vi "test request state rounds.vi"(8 "error in (no error)":errorcluster) -> (0 "error out":errorcluster, 3 "body":string)   [LabVIEW 2020, in "MCP Server tests.lvlib"]
doc: "Multi round-trip requests of MCP 2026-07-28 with requestState. fake_tool_two_questions asks the key first (Ask User.vi, a name) and in a later round the key second (Confirm With User.vi). Round 1 (id 70) is answered input_required with inputRequests.first and a requestState mcp-rs-...; round 2 (id 701) sends inputResponses first accept name Ada with that requestState and is answered input_required with inputRequests.second and a new requestState; round 3 (id 702) sends only the answer to second with the new requestState - the server carries the answer to first across the rounds - and the result is complete with name Ada and stored TRUE. The requests are sent with the LabVIEW HTTP Client directly."
uses:
  MCP Server tests.lvlib
  <vilib>/JDP Science/JSONtext/Next JSON Value.vi
  <vilib>/JDP Science/JSONtext/String Subset.vi
  <vilib>/JDP Science/JSONtext/Parsing/Advance past next JSON Value (inlined COPY).vi
  <vilib>/JDP Science/JSONtext/Parsing/Advance past whitespace.vi
  <vilib>/JDP Science/JSONtext/Parsing/Advance past String.vi
  <vilib>/JDP Science/JSONtext/Parsing/Advance past Number.vi
  <vilib>/JDP Science/JSONtext/Parsing/Advance past Line Ending.vi
  <vilib>/JDP Science/JSONtext/Parsing/Parse Full Path or Item Name.vi
  <vilib>/JDP Science/JSONtext/Parsing/Advance past Array.vi
  <vilib>/JDP Science/JSONtext/Parsing/Advance past Object.vi
  <vilib>/JDP Science/JSONtext/support/Error Cluster From Code.vi
  <vilib>/JDP Science/JSONtext/Offset/Find Item Locations by Path.vi
  <vilib>/addons/_JKI Toolkits/Caraya/classes/Test/Test.lvclass
  <vilib>/JDP Science/JSONtext/JSONtext.lvlib
  <vilib>/addons/_JKI Toolkits/Caraya/classes/Assert/Assert.lvclass
panel:
  out "lookup error":errorcluster
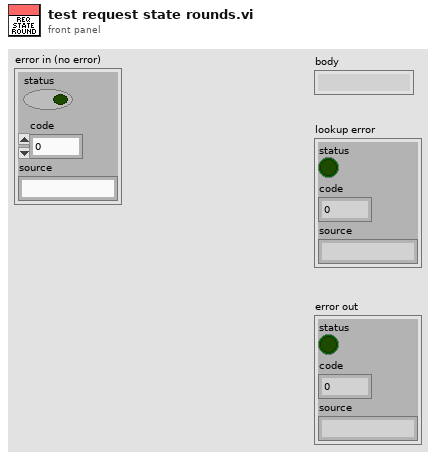
[diagram p1: front panel]
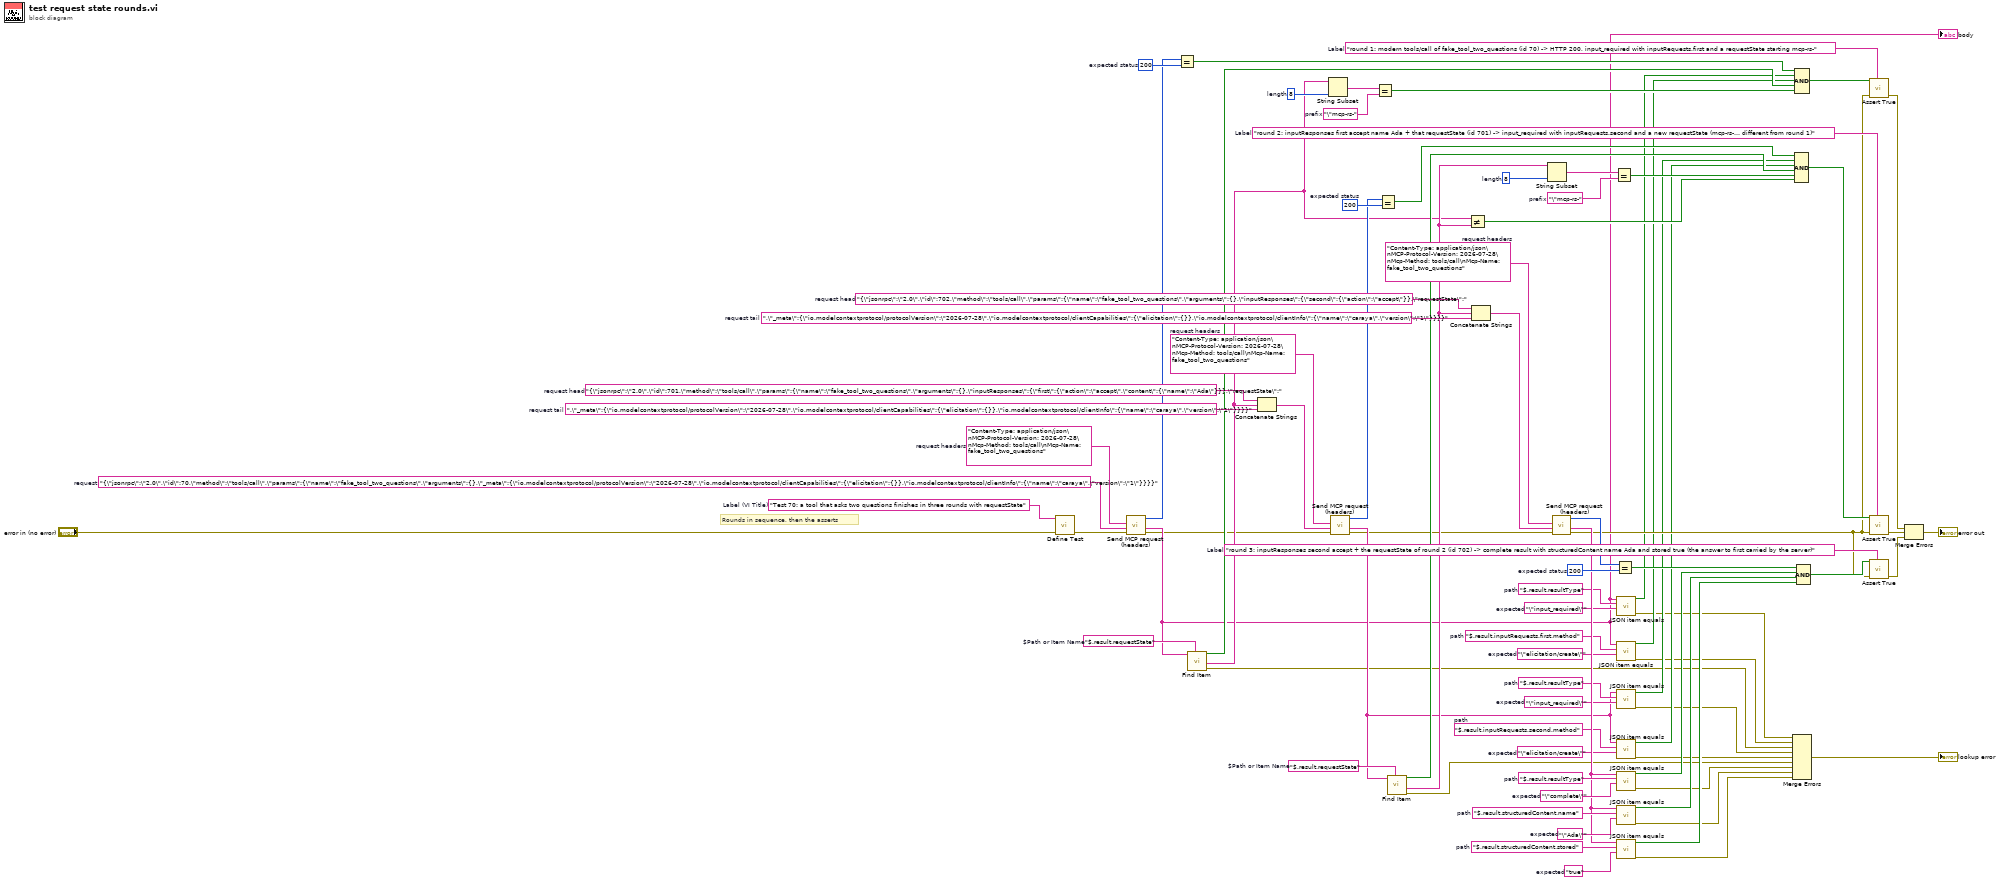
[diagram p0: block diagram]
diagram:
  w81 = "round 3: inputResponses second accept + the requestState of round 2 (id 702) -> complete result with structuredContent name Ada and stored true (the answer to first carried by the server)"  # Label
  w78 = "round 2: inputResponses first accept name Ada + that requestState (id 701) -> input_required with inputRequests.second and a new requestState (mcp-rs-… different from round 1)"  # Label
  w75 = "round 1: modern tools/call of fake_tool_two_questions (id 70) -> HTTP 200, input_required with inputRequests.first and a requestState starting mcp-rs-"  # Label
  w71 = "true"  # expected
  w70 = "$.result.structuredContent.stored"  # path
  w67 = "\"Ada\""  # expected
  w66 = "$.result.structuredContent.name"  # path
  w63 = "\"complete\""  # expected
  w62 = "$.result.resultType"  # path
  w60 = 200  # expected status
  w56 = "Content-Type: application/json\nMCP-Protocol-Version: 2026-07-28\nMcp-Method: tools/call\nMcp-Name: fake_tool_two_questions"  # request headers
  w54 = ",\"_meta\":{\"io.modelcontextprotocol/protocolVersion\":\"2026-07-28\",\"io.modelcontextprotocol/clientCapabilities\":{\"elicitation\":{}},\"io.modelcontextprotocol/clientInfo\":{\"name\":\"caraya\",\"version\":\"1\"}}}}"  # request tail
  w53 = "{\"jsonrpc\":\"2.0\",\"id\":702,\"method\":\"tools/call\",\"params\":{\"name\":\"fake_tool_two_questions\",\"arguments\":{},\"inputResponses\":{\"second\":{\"action\":\"accept\"}},\"requestState\":"  # request head
  w49 = 8  # length
  w48 = "\"mcp-rs-"  # prefix
  w44 = "$.result.requestState"  # $Path or Item Name
  w41 = "\"elicitation/create\""  # expected
  w40 = "$.result.inputRequests.second.method"  # path
  w37 = "\"input_required\""  # expected
  w36 = "$.result.resultType"  # path
  w34 = 200  # expected status
  w30 = "Content-Type: application/json\nMCP-Protocol-Version: 2026-07-28\nMcp-Method: tools/call\nMcp-Name: fake_tool_two_questions"  # request headers
  w28 = ",\"_meta\":{\"io.modelcontextprotocol/protocolVersion\":\"2026-07-28\",\"io.modelcontextprotocol/clientCapabilities\":{\"elicitation\":{}},\"io.modelcontextprotocol/clientInfo\":{\"name\":\"caraya\",\"version\":\"1\"}}}}"  # request tail
  w27 = "{\"jsonrpc\":\"2.0\",\"id\":701,\"method\":\"tools/call\",\"params\":{\"name\":\"fake_tool_two_questions\",\"arguments\":{},\"inputResponses\":{\"first\":{\"action\":\"accept\",\"content\":{\"name\":\"Ada\"}}},\"requestState\":"  # request head
  w24 = 8  # length
  w23 = "\"mcp-rs-"  # prefix
  w19 = "$.result.requestState"  # $Path or Item Name
  w16 = "\"elicitation/create\""  # expected
  w15 = "$.result.inputRequests.first.method"  # path
  w12 = "\"input_required\""  # expected
  w11 = "$.result.resultType"  # path
  w9 = 200  # expected status
  w5 = "Content-Type: application/json\nMCP-Protocol-Version: 2026-07-28\nMcp-Method: tools/call\nMcp-Name: fake_tool_two_questions"  # request headers
  w4 = "{\"jsonrpc\":\"2.0\",\"id\":70,\"method\":\"tools/call\",\"params\":{\"name\":\"fake_tool_two_questions\",\"arguments\":{},\"_meta\":{\"io.modelcontextprotocol/protocolVersion\":\"2026-07-28\",\"io.modelcontextprotocol/clientCapabilities\":{\"elicitation\":{}},\"io.modelcontextprotocol/clientInfo\":{\"name\":\"caraya\",\"version\":\"1\"}}}}"  # request
  w2 = "Test 70: a tool that asks two questions finishes in three rounds with requestState"  # Label (VI Title)
  # "Rounds in sequence, then the asserts"
  n1 = call <vilib>:"Define Test.vi"("error in (no error)"="error in (no error)", "Label (VI Title)"=w2) -> ("error out"=w3:errorcluster)  [unwired: 8 in, 1 out]
  n2 = call "Send MCP request (headers).vi"("error in (no error)"=w3, "request"=w4, "request headers"=w5) -> ("error out"=w6:errorcluster, "response"=w7:string, "status code"=w8:i32)  [unwired: 5 in, 1 out]
  "body" <- w7
  n3 = Equal?(x=w8, y=w9) -> (x = y?=w10:bool)
  n4 = call <vilib>:"Find Item.vi"("$Path or Item Name"=w19, "JSON"=w7) -> ("error out"=w20:errorcluster, "<JSON>"=w21:string, "Found"=w22:bool)  [unwired: 6 in, 1 out]
  n5 = Concatenate Strings(w27, w21, w28) -> (w29:string)
  n6 = String Subset(string=w21, length (rest)=w24) -> (substring=w25:string)  [unwired: 1 in]
  n7 = call "Send MCP request (headers).vi"("error in (no error)"=w6, "request"=w29, "request headers"=w30) -> ("error out"=w31:errorcluster, "response"=w32:string, "status code"=w33:i32)  [unwired: 5 in, 1 out]
  n8 = Equal?(x=w25, y=w23) -> (x = y?=w26:bool)
  n9 = Equal?(x=w33, y=w34) -> (x = y?=w35:bool)
  n10 = call <vilib>:"Find Item.vi"("$Path or Item Name"=w44, "JSON"=w32) -> ("error out"=w45:errorcluster, "<JSON>"=w46:string, "Found"=w47:bool)  [unwired: 6 in, 1 out]
  n11 = Not Equal?(x=w21, y=w46) -> (x != y?=w52:bool)
  n12 = Concatenate Strings(w53, w46, w54) -> (w55:string)
  n13 = String Subset(string=w46, length (rest)=w49) -> (substring=w50:string)  [unwired: 1 in]
  n14 = call "Send MCP request (headers).vi"("error in (no error)"=w31, "request"=w55, "request headers"=w56) -> ("error out"=w57:errorcluster, "response"=w58:string, "status code"=w59:i32)  [unwired: 5 in, 1 out]
  n15 = Equal?(x=w50, y=w48) -> (x = y?=w51:bool)
  n16 = Equal?(x=w59, y=w60) -> (x = y?=w61:bool)
  n17 = call "JSON item equals.vi"("expected"=w12, "path"=w11, "JSON"=w7) -> ("error out"=w13:errorcluster, "equal?"=w14:bool)  [unwired: 6 in, 1 out]
  n18 = call "JSON item equals.vi"("expected"=w16, "path"=w15, "JSON"=w7) -> ("error out"=w17:errorcluster, "equal?"=w18:bool)  [unwired: 6 in, 1 out]
  n19 = call "JSON item equals.vi"("expected"=w37, "path"=w36, "JSON"=w32) -> ("error out"=w38:errorcluster, "equal?"=w39:bool)  [unwired: 6 in, 1 out]
  n20 = call "JSON item equals.vi"("expected"=w41, "path"=w40, "JSON"=w32) -> ("error out"=w42:errorcluster, "equal?"=w43:bool)  [unwired: 6 in, 1 out]
  n21 = call "JSON item equals.vi"("expected"=w63, "path"=w62, "JSON"=w58) -> ("error out"=w64:errorcluster, "equal?"=w65:bool)  [unwired: 6 in, 1 out]
  n22 = call "JSON item equals.vi"("expected"=w67, "path"=w66, "JSON"=w58) -> ("error out"=w68:errorcluster, "equal?"=w69:bool)  [unwired: 6 in, 1 out]
  n23 = call "JSON item equals.vi"("expected"=w71, "path"=w70, "JSON"=w58) -> ("error out"=w72:errorcluster, "equal?"=w73:bool)  [unwired: 6 in, 1 out]
  n24 = Merge Errors(w13, w17, w20, w38, w42, w45, w64, w68, w72) -> (→"lookup error":errorcluster)
  n25 = Compound Arithmetic op=AND(w35, w39, w43, w47, w51, w52) -> (w77:bool)
  n26 = Compound Arithmetic op=AND(w10, w14, w18, w22, w26) -> (w74:bool)
  n27 = Compound Arithmetic op=AND(w61, w65, w69, w73) -> (w80:bool)
  n28 = call <vilib>:"Assert True.vi"("Label"=w75, "error in (no error)"=w57, "True?"=w74) -> ("error out"=w76:errorcluster)  [unwired: 7 in, 1 out]
  n29 = call <vilib>:"Assert True.vi"("Label"=w78, "error in (no error)"=w57, "True?"=w77) -> ("error out"=w79:errorcluster)  [unwired: 7 in, 1 out]
  n30 = call <vilib>:"Assert True.vi"("Label"=w81, "error in (no error)"=w57, "True?"=w80) -> ("error out"=w82:errorcluster)  [unwired: 7 in, 1 out]
  n31 = Merge Errors(w76, w79, w82) -> (→"error out":errorcluster)
